vi "read_Float.vi"(8 "错误输入（无错误）":errorcluster, 10 "Address":string, 11 "URL":string="opc://localhost/National Instruments.NIOPCServers.V5/Channel1.Battery_Testing.") -> (0 "error out":errorcluster caption="错误输出", 2 "Value":dbl, 3 "ok?":bool)   [LabVIEW 2013]
panel:
  out "数据":u16
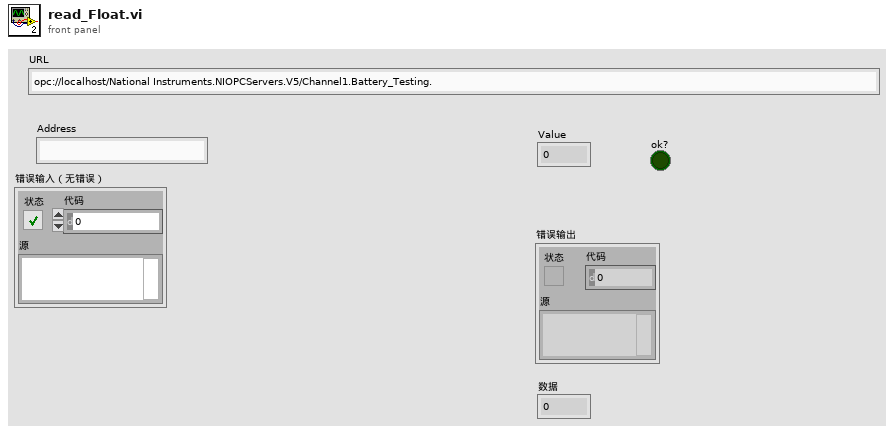
[diagram p1: front panel]
types:
  T1 = enum16{"Read", "Write", "ReadWrite", "BufferedRead", "BufferedReadWrite"}
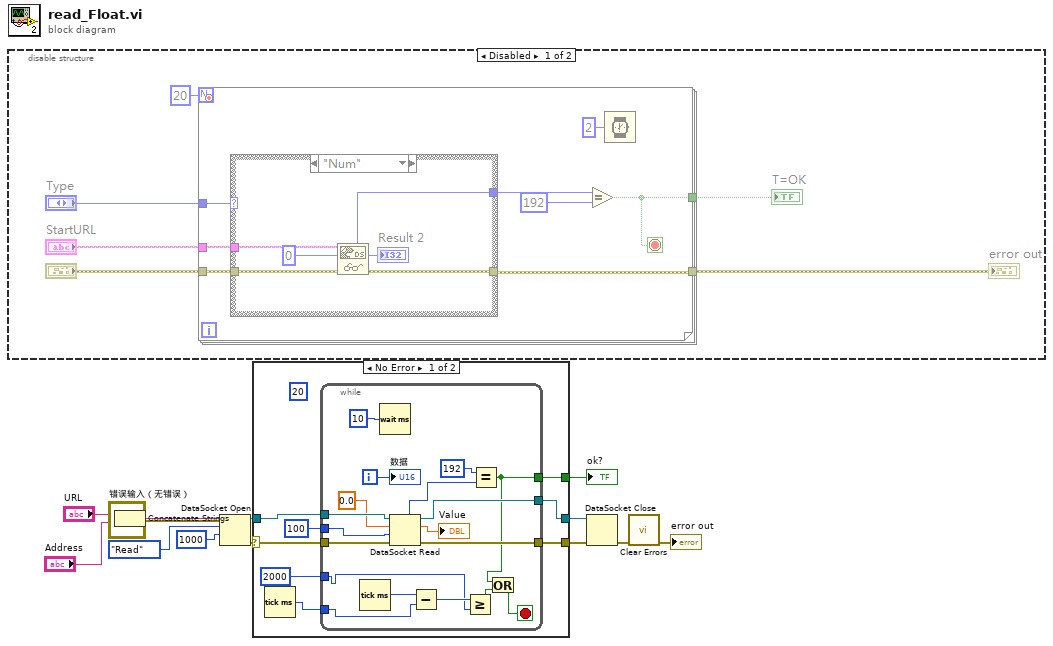
[diagram p0: block diagram]
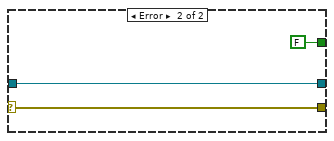
[diagram p3: hidden frame]
diagram:
  n1 = disable-structure shown="Disabled" {
    frame Disabled {
    }
    frame Enabled {
    }
  }
  n2 = Concatenate Strings("URL", "Address") -> (w11:string)
  n3 = DataSocket Open(8:"错误输入（无错误）", 9:1000 ("毫秒超时(10000)"), 10:T1."Read" ("模式"), 11:w11) -> (0:w3:errorcluster, 3:w8:refnum<k13>)
  n4 = case shown="No Error" w3 {
    selector: w3 -> [w17 w40]
    tunnel: w8 -> [w20 w42]
    tunnel: [w19 w42] -> w7
    tunnel: [w18 w40] -> w6
    tunnel: [w16 FALSE ("timed out")] -> w2
    frame No Error {
      (unwired) 20
      n5 = Tick Count (ms)() -> (millisecond timer value=w15:u32)
      n6 = while {
        tunnel: 100 ("毫秒超时(0)") -> [w38]
        tunnel: w17 -> [w37]
        tunnel: w20 -> [w36]
        tunnel: [w35] -> w19
        tunnel: [w34] -> w18
        tunnel: [w23] -> w16
        tunnel: w15 -> [w25]
        tunnel: 2000 ("毫秒超时(0)") -> [w24]
        i -> [w33]
        stop <- w22 stop-if-true
        n7 = Tick Count (ms)() -> (millisecond timer value=w26:u32)
        n8 = Wait (ms)(milliseconds to wait=u32 10 ("等待时间（毫秒）")) -> ()  [unwired: 1 out]
        n9 = DataSocket Read(8:w37, 9:w38, 10:0.0 ("Value"), 11:w36) -> (0:w34:errorcluster, 2:→"Value":dbl, 3:w35:refnum<k13>, 5:w32:u64)  [unwired: 1 in, 3 out]
        n10 = Subtract(x=w26, y=w25) -> (x-y=w27:u32)
        n11 = Greater Or Equal?(x=w27, y=w24) -> (x >= y?=w28:bool)
        n12 = Equal?(x=u64 192, y=w32) -> (x = y?=w23:bool)
        n13 = Or(x=w23, y=w28) -> (x .or. y?=w22:bool)
        "数据" <- w33
      }
    }
    frame Error {
    }
  }
  "ok?" <- w2
  n14 = DataSocket Close(8:w6, 11:w7) -> (0:w5:errorcluster)  [unwired: 1 in, 1 out]
  n15 = call <vilib>:"Clear Errors.vi"("error in (no error)"=w5) -> ("error out"=→"error out":errorcluster)  [unwired: 6 in]
